vi "Lock-in_dem_mul.vi"(3 "Phase&Tc":T1(array[cluster])=[{"Phase"=-4.587448254233148, "Time constant"=0.10000000000000009, "Set TimeConstant"=FALSE, "Autophase"=FALSE, "Order"=2.0}, {"Phase"=0.0, "Time constant"=0.2, "Set TimeConstant"=FALSE, "Autophase"=FALSE, "Order"=2.0}, {"Phase"=0.0, "Time constant"=0.0, "Set TimeConstant"=FALSE, "Autophase"=FALSE, "Order"=0.0}, {"Phase"=0.0, "Time constant"=0.0, "Set TimeConstant"=FALSE, "Autophase"=FALSE, "Order"=0.0}] {"Phase" min=0.0 max=360.0 scale=0.0..360.0}, 4 "Ref in":T2(array[cluster])=[{"Ref X"=array[40000 elements], "Ref Y"=array[40000 elements], "AI Rate"=200000.0, "AI Block Size"=40000.0, "Frequency"=20.0, "Ref amp"=5.0}, {"Ref X"=array[40000 elements], "Ref Y"=array[40000 elements], "AI Rate"=200000.0, "AI Block Size"=40000.0, "Frequency"=20.0, "Ref amp"=5.0}, {"Ref X"=array[40000 elements], "Ref Y"=array[40000 elements], "AI Rate"=200000.0, "AI Block Size"=40000.0, "Frequency"=20.0, "Ref amp"=5.0}, {"Ref X"=array[40000 elements], "Ref Y"=array[40000 elements], "AI Rate"=200000.0, "AI Block Size"=40000.0, "Frequency"=20.0, "Ref amp"=5.0}] {"Ref amp" step=0.001 format="%0.4f"; "Frequency" step=0.001 format="%0.4f"; "AI Block Size" step=0.001 format="%0.4f"; "AI Rate" step=0.001 format="%0.4f"}, 5 "Signal":dbl[][](array[numeric])=array4x40000[160000 elements]) -> (1 "Demodulation":dbl[][](array[numeric])=[[0.032308985716257205, -0.0020089800684537727, 0.032371384878394444, -3.5583001590229886], [0.023385861272623584, -0.0014539178662531169, 0.02343101330770514, -3.5574201885889787], [-3.111140914765216e-05, 2.7289487058700542e-06, 3.123206852318323e-05, -5.0131650508604935], [-3.1370210865590166e-05, 3.1631661467659442e-06, 3.1532606636697875e-05, -5.751181571584788]])   [LabVIEW 2011]
uses:
  <vilib>/Analysis/3filter.llb/Filter Passband Type.ctl
  <vilib>/Analysis/NI_AALBase.lvlib
  <vilib>/ptbypt/NI_PtbyPt.lvlib
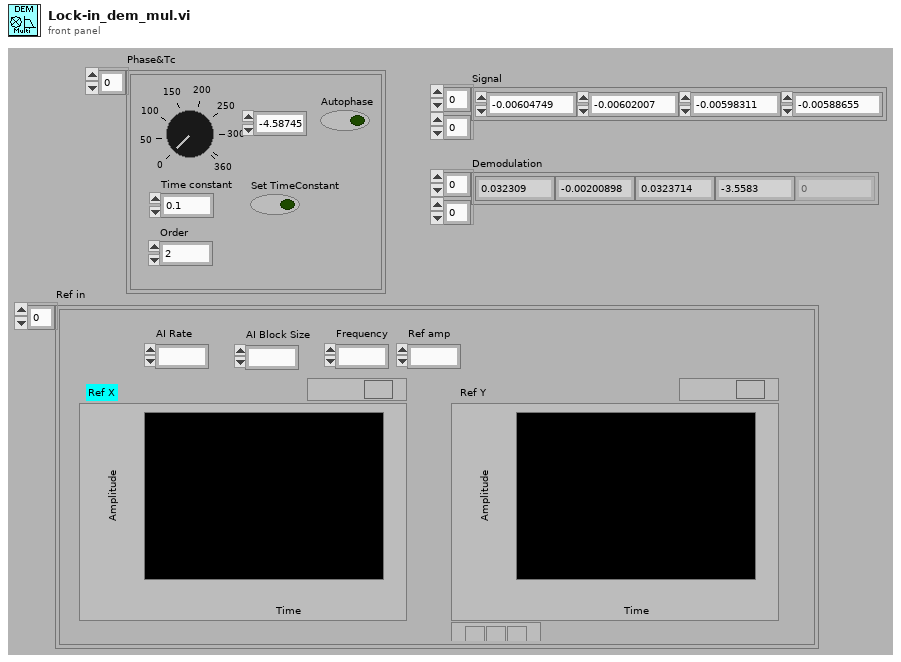
[diagram p1: front panel]
types:
  T1 = cluster{"Phase":dbl, "Time constant":dbl, "Set TimeConstant":bool, "Autophase":bool, "Order":dbl}[]
  T2 = cluster{"Ref X":dbl[], "Ref Y":dbl[], "AI Rate":dbl, "AI Block Size":dbl, "Frequency":dbl, "Ref amp":dbl}[]
  T3 = typedef "NI_AALBase.lvlib/Filter Passband Type.ctl" = enum32{"Lowpass", "Highpass", "Bandpass", "Bandstop"}
  T4 = cluster{"Ref X":dbl[], "Ref Y":dbl[], "AI Rate":dbl, "AI Block Size":dbl, "Frequency":dbl, "Ref amp":dbl}
  T5 = cluster{"Phase":dbl, "Time constant":dbl, "Set TimeConstant":bool, "Autophase":bool, "Order":dbl}
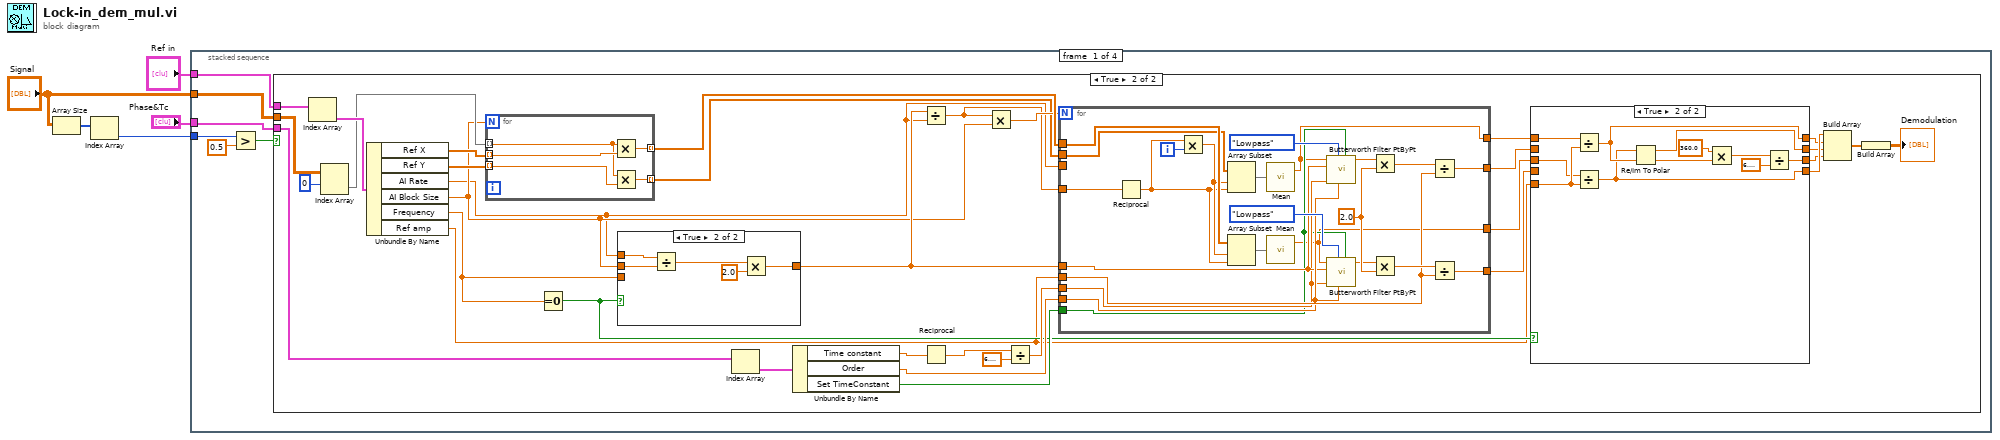
[diagram p0: block diagram]
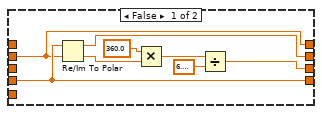
[diagram p3: hidden frame]
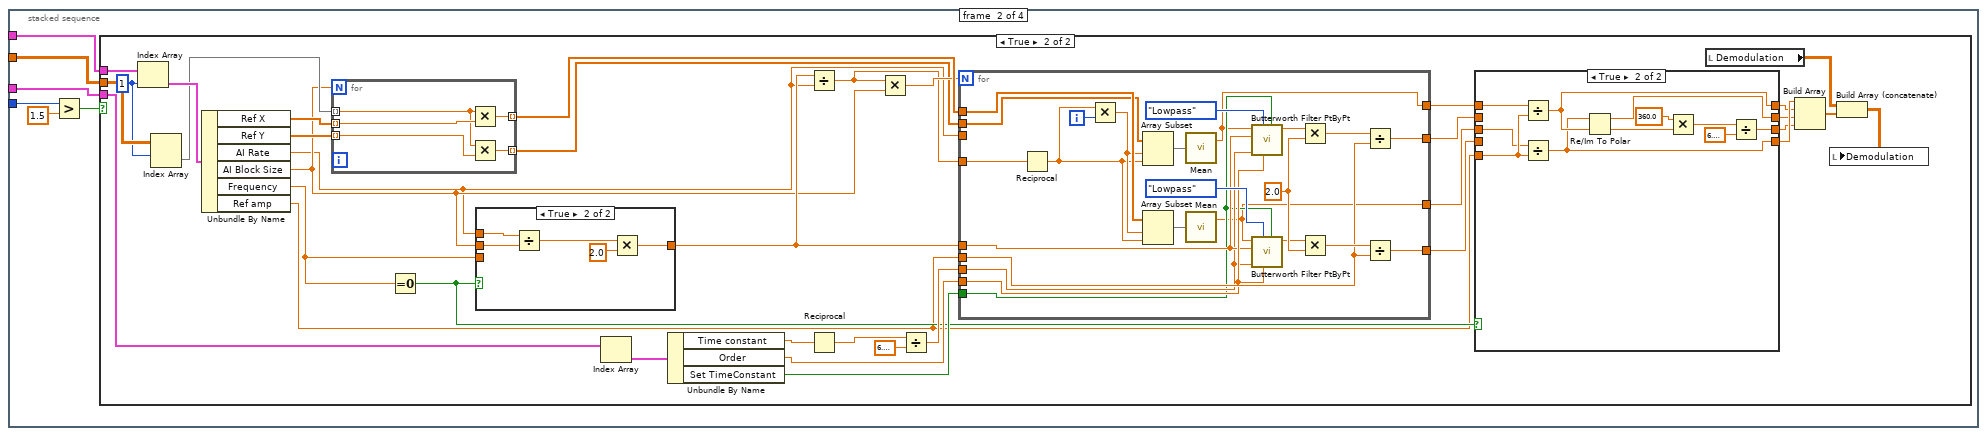
[diagram p5: hidden frame]
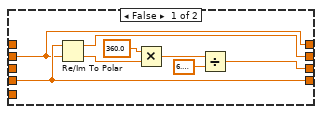
[diagram p7: hidden frame]
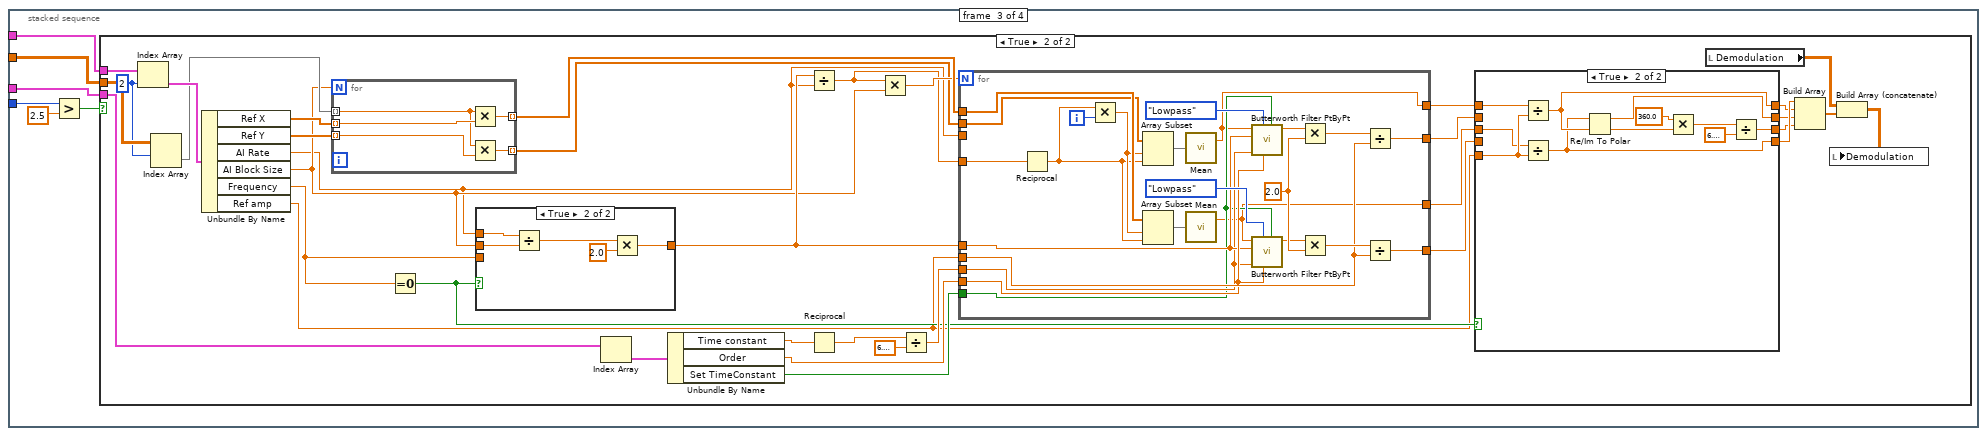
[diagram p9: hidden frame]
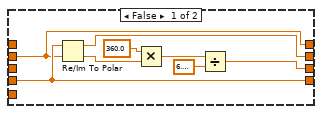
[diagram p11: hidden frame]
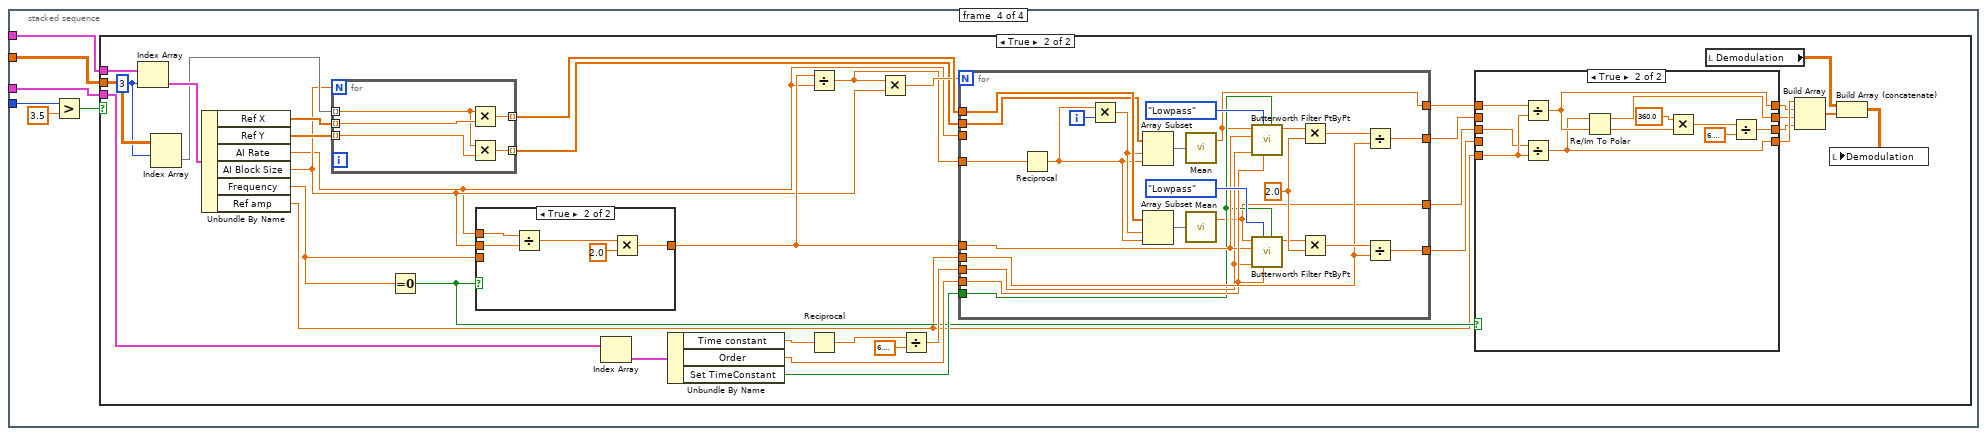
[diagram p13: hidden frame]
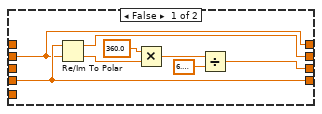
[diagram p15: hidden frame]
diagram:
  n1 = Array Size(array="Signal") -> (size(s)=w2:i32[])
  n2 = Index Array(array=w2) -> (element=w1:i32)  [unwired: 1 in]
  n3 = stacked-sequence {
    tunnel: "Signal" -> [w11 w106 w202 w298]
    tunnel: "Ref in" -> [w10 w105 w201 w297]
    tunnel: "Phase&Tc" -> [w9 w104 w200 w296]
    tunnel: w1 -> [w6 w101 w197 w293]
    frame #0 {
      n4 = Greater?(x=w6, y=0.5) -> (0:w8:bool)
      n5 = case shown="True" w8 {
        tunnel: w11 -> [_ w35]
        tunnel: w10 -> [_ w34]
        tunnel: w9 -> [_ w32]
        frame False {
        }
        frame True {
          n6 = Index Array(array=w34) -> (element=w33:T4)  [unwired: 1 in]
          n7 = Index Array(array=w35, index (row)=0) -> (element=w29:dbl[])  [unwired: 1 in]
          n8 = Unbundle By Name(w33) -> ("Ref X"=w39:dbl[], "Ref Y"=w38:dbl[], "AI Rate"=w24:dbl, "AI Block Size"=w25:dbl, "Frequency"=w27:dbl, "Ref amp"=w12:dbl)
          n9 = for {
            N: w25 -> [_]
            tunnel: w29 -> [w98] mode=indexing
            tunnel: w39 -> [w100] mode=indexing
            tunnel: [w99] -> w46 mode=indexing
            tunnel: w38 -> [w97] mode=indexing
            tunnel: [w96] -> w43 mode=indexing
            n10 = Multiply(x=w98, y=w100) -> (x*y=w99:dbl)
            n11 = Multiply(x=w98, y=w97) -> (x*y=w96:dbl)
          }
          n12 = Equal To 0?(x=w27) -> (x = 0?=w23:bool)
          n13 = case shown="True" w23 {
            tunnel: w27 -> [w66 _]
            tunnel: [w66 w67] -> w26
            tunnel: w25 -> [_ w71]
            tunnel: w24 -> [_ w70]
            frame False {
            }
            frame True {
              n14 = Divide(x=w70, y=w71) -> (x/y=w69:dbl)
              n15 = Multiply(x=w69, y=2.0) -> (x*y=w67:dbl)
            }
          }
          n16 = Index Array(array=w32) -> (element=w31:T5)  [unwired: 1 in]
          n17 = Unbundle By Name(w31) -> ("Time constant"=w37:dbl, "Order"=w36:dbl, "Set TimeConstant"=w30:bool)
          n18 = Divide(x=w26, y=w24) -> (x/y=w44:dbl)
          n19 = Reciprocal(x=w37) -> (1/x=w42:dbl)
          n20 = Multiply(x=w44, y=w25) -> (x*y=w45:dbl)
          n21 = Divide(x=w42, y=6.283185307179586) -> (x/y=w40:dbl)
          n22 = for {
            N: w45 -> [_]
            tunnel: w24 -> [_]
            tunnel: w46 -> [w95]
            tunnel: w44 -> [w88]
            tunnel: w43 -> [w93]
            tunnel: w40 -> [w78]
            tunnel: w12 -> [w81]
            tunnel: w36 -> [w80]
            tunnel: w26 -> [w79]
            tunnel: w30 -> [w77]
            tunnel: [w75] -> w22
            tunnel: [w74] -> w21
            tunnel: [w73] -> w20
            tunnel: [w72] -> w19
            i -> [w94]
            w83 = 2.0 ("y")
            n23 = Reciprocal(x=w88) -> (1/x=w91:dbl)
            n24 = Multiply(x=w91, y=w94) -> (x*y=w92:dbl)
            n25 = Array Subset(array=w93, index=w92, length=w91) -> (w89:dbl[])
            n26 = Array Subset(array=w95, index=w92, length=w91) -> (w90:dbl[])
            n27 = call <vilib>:"Mean.vi"("X"=w89) -> ("mean"=w72:dbl)  [unwired: 1 out]
            n28 = call <vilib>:"Mean.vi"("X"=w90) -> ("mean"=w73:dbl)  [unwired: 1 out]
            n29 = call <vilib>:"Butterworth Filter PtByPt.vi"("initialize"=w77, "order"=w80, "filter type"=Filter_Passband_Type."Lowpass", "low cutoff freq: fl"=w78, "sampling freq: fs"=w79, "x"=w72) -> ("Filtered x"=w84:dbl)  [unwired: 3 in, 1 out]
            n30 = call <vilib>:"Butterworth Filter PtByPt.vi"("initialize"=w77, "order"=w80, "filter type"=Filter_Passband_Type."Lowpass", "low cutoff freq: fl"=w78, "sampling freq: fs"=w79, "x"=w73) -> ("Filtered x"=w76:dbl)  [unwired: 3 in, 1 out]
            n31 = Multiply(x=w84, y=w83) -> (x*y=w82:dbl)
            n32 = Multiply(x=w76, y=w83) -> (x*y=w85:dbl)
            n33 = Divide(x=w82, y=w81) -> (x/y=w74:dbl)
            n34 = Divide(x=w85, y=w81) -> (x/y=w75:dbl)
          }
          n35 = case shown="True" w23 {
            tunnel: w22 -> [w50 _]
            tunnel: w21 -> [w49 _]
            tunnel: w20 -> [_ w58]
            tunnel: w19 -> [_ w59]
            tunnel: [w50 w56] -> w18
            tunnel: [w49 w57] -> w17
            tunnel: [w48 w62] -> w16
            tunnel: [w47 w55] -> w15
            tunnel: w12 -> [_ w60]
            frame False {
              n36 = Re/Im To Polar(2:w49, 3:w50) -> (0:w54:dbl, 1:w48:dbl)
              n37 = Multiply(x=360.0 ("y"), y=w54) -> (x*y=w51:dbl)
              n38 = Divide(x=w51, y=6.283185307179586) -> (x/y=w47:dbl)
            }
            frame True {
              n39 = Divide(x=w59, y=w60) -> (x/y=w57:dbl)
              n40 = Divide(x=w58, y=w60) -> (x/y=w56:dbl)
              n41 = Re/Im To Polar(2:w57, 3:w56) -> (0:w61:dbl, 1:w62:dbl)
              n42 = Multiply(x=360.0 ("y"), y=w61) -> (x*y=w63:dbl)
              n43 = Divide(x=w63, y=6.283185307179586) -> (x/y=w55:dbl)
            }
          }
          n44 = Build Array(w18, w17, w16, w15) -> (w14:dbl[])
          n45 = Build Array(w14) -> (→"Demodulation":dbl[][])
        }
      }
    }
    frame #1 {
      n46 = Greater?(x=w101, y=1.5) -> (0:w103:bool)
      n47 = case shown="True" w103 {
        tunnel: w106 -> [_ w131]
        tunnel: w105 -> [_ w130]
        tunnel: w104 -> [_ w128]
        frame False {
        }
        frame True {
          w109 = 1 ("index")
          n48 = Index Array(array=w130, index=w109) -> (element=w129:T4)
          n49 = Index Array(array=w131, index (row)=w109) -> (element=w125:dbl[])  [unwired: 1 in]
          n50 = Unbundle By Name(w129) -> ("Ref X"=w135:dbl[], "Ref Y"=w134:dbl[], "AI Rate"=w121:dbl, "AI Block Size"=w122:dbl, "Frequency"=w124:dbl, "Ref amp"=w110:dbl)
          n51 = for {
            N: w122 -> [_]
            tunnel: w125 -> [w194] mode=indexing
            tunnel: w135 -> [w196] mode=indexing
            tunnel: [w195] -> w142 mode=indexing
            tunnel: w134 -> [w193] mode=indexing
            tunnel: [w192] -> w139 mode=indexing
            n52 = Multiply(x=w194, y=w196) -> (x*y=w195:dbl)
            n53 = Multiply(x=w194, y=w193) -> (x*y=w192:dbl)
          }
          n54 = Equal To 0?(x=w124) -> (x = 0?=w120:bool)
          n55 = case shown="True" w120 {
            tunnel: w124 -> [w162 _]
            tunnel: [w162 w163] -> w123
            tunnel: w122 -> [_ w167]
            tunnel: w121 -> [_ w166]
            frame False {
            }
            frame True {
              n56 = Divide(x=w166, y=w167) -> (x/y=w165:dbl)
              n57 = Multiply(x=w165, y=2.0) -> (x*y=w163:dbl)
            }
          }
          n58 = Index Array(array=w128) -> (element=w127:T5)  [unwired: 1 in]
          n59 = Unbundle By Name(w127) -> ("Time constant"=w133:dbl, "Order"=w132:dbl, "Set TimeConstant"=w126:bool)
          n60 = Divide(x=w123, y=w121) -> (x/y=w140:dbl)
          n61 = Reciprocal(x=w133) -> (1/x=w138:dbl)
          n62 = Multiply(x=w140, y=w122) -> (x*y=w141:dbl)
          n63 = Divide(x=w138, y=6.283185307179586) -> (x/y=w136:dbl)
          n64 = for {
            N: w141 -> [_]
            tunnel: w121 -> [_]
            tunnel: w142 -> [w191]
            tunnel: w140 -> [w184]
            tunnel: w139 -> [w189]
            tunnel: w136 -> [w174]
            tunnel: w110 -> [w177]
            tunnel: w132 -> [w176]
            tunnel: w123 -> [w175]
            tunnel: w126 -> [w173]
            tunnel: [w171] -> w119
            tunnel: [w170] -> w118
            tunnel: [w169] -> w117
            tunnel: [w168] -> w116
            i -> [w190]
            w179 = 2.0 ("y")
            n65 = Reciprocal(x=w184) -> (1/x=w187:dbl)
            n66 = Multiply(x=w187, y=w190) -> (x*y=w188:dbl)
            n67 = Array Subset(array=w189, index=w188, length=w187) -> (w185:dbl[])
            n68 = Array Subset(array=w191, index=w188, length=w187) -> (w186:dbl[])
            n69 = call <vilib>:"Mean.vi"("X"=w185) -> ("mean"=w168:dbl)  [unwired: 1 out]
            n70 = call <vilib>:"Mean.vi"("X"=w186) -> ("mean"=w169:dbl)  [unwired: 1 out]
            n71 = call <vilib>:"Butterworth Filter PtByPt.vi"("initialize"=w173, "order"=w176, "filter type"=Filter_Passband_Type."Lowpass", "low cutoff freq: fl"=w174, "sampling freq: fs"=w175, "x"=w168) -> ("Filtered x"=w180:dbl)  [unwired: 3 in, 1 out]
            n72 = call <vilib>:"Butterworth Filter PtByPt.vi"("initialize"=w173, "order"=w176, "filter type"=Filter_Passband_Type."Lowpass", "low cutoff freq: fl"=w174, "sampling freq: fs"=w175, "x"=w169) -> ("Filtered x"=w172:dbl)  [unwired: 3 in, 1 out]
            n73 = Multiply(x=w180, y=w179) -> (x*y=w178:dbl)
            n74 = Multiply(x=w172, y=w179) -> (x*y=w181:dbl)
            n75 = Divide(x=w178, y=w177) -> (x/y=w170:dbl)
            n76 = Divide(x=w181, y=w177) -> (x/y=w171:dbl)
          }
          n77 = case shown="True" w120 {
            tunnel: w119 -> [w146 _]
            tunnel: w118 -> [w145 _]
            tunnel: w117 -> [_ w154]
            tunnel: w116 -> [_ w155]
            tunnel: [w146 w152] -> w115
            tunnel: [w145 w153] -> w114
            tunnel: [w144 w158] -> w113
            tunnel: [w143 w151] -> w112
            tunnel: w110 -> [_ w156]
            frame False {
              n78 = Re/Im To Polar(2:w145, 3:w146) -> (0:w150:dbl, 1:w144:dbl)
              n79 = Multiply(x=360.0 ("y"), y=w150) -> (x*y=w147:dbl)
              n80 = Divide(x=w147, y=6.283185307179586) -> (x/y=w143:dbl)
            }
            frame True {
              n81 = Divide(x=w155, y=w156) -> (x/y=w153:dbl)
              n82 = Divide(x=w154, y=w156) -> (x/y=w152:dbl)
              n83 = Re/Im To Polar(2:w153, 3:w152) -> (0:w157:dbl, 1:w158:dbl)
              n84 = Multiply(x=360.0 ("y"), y=w157) -> (x*y=w159:dbl)
              n85 = Divide(x=w159, y=6.283185307179586) -> (x/y=w151:dbl)
            }
          }
          n86 = local read "Demodulation"() -> (w108:dbl[][])
          n87 = Build Array(w115, w114, w113, w112) -> (w111:dbl[])
          n88 = Build Array (concatenate)(w108, w111) -> (w107:dbl[][])
          n89 = local write "Demodulation"(w107) -> ()
        }
      }
    }
    frame #2 {
      n90 = Greater?(x=w197, y=2.5) -> (0:w199:bool)
      n91 = case shown="True" w199 {
        tunnel: w202 -> [_ w227]
        tunnel: w201 -> [_ w226]
        tunnel: w200 -> [_ w224]
        frame False {
        }
        frame True {
          w205 = 2 ("index")
          n92 = Index Array(array=w226, index=w205) -> (element=w225:T4)
          n93 = Index Array(array=w227, index (row)=w205) -> (element=w221:dbl[])  [unwired: 1 in]
          n94 = Unbundle By Name(w225) -> ("Ref X"=w231:dbl[], "Ref Y"=w230:dbl[], "AI Rate"=w217:dbl, "AI Block Size"=w218:dbl, "Frequency"=w220:dbl, "Ref amp"=w206:dbl)
          n95 = for {
            N: w218 -> [_]
            tunnel: w221 -> [w290] mode=indexing
            tunnel: w231 -> [w292] mode=indexing
            tunnel: [w291] -> w238 mode=indexing
            tunnel: w230 -> [w289] mode=indexing
            tunnel: [w288] -> w235 mode=indexing
            n96 = Multiply(x=w290, y=w292) -> (x*y=w291:dbl)
            n97 = Multiply(x=w290, y=w289) -> (x*y=w288:dbl)
          }
          n98 = Equal To 0?(x=w220) -> (x = 0?=w216:bool)
          n99 = case shown="True" w216 {
            tunnel: w220 -> [w258 _]
            tunnel: [w258 w259] -> w219
            tunnel: w218 -> [_ w263]
            tunnel: w217 -> [_ w262]
            frame False {
            }
            frame True {
              n100 = Divide(x=w262, y=w263) -> (x/y=w261:dbl)
              n101 = Multiply(x=w261, y=2.0) -> (x*y=w259:dbl)
            }
          }
          n102 = Index Array(array=w224) -> (element=w223:T5)  [unwired: 1 in]
          n103 = Unbundle By Name(w223) -> ("Time constant"=w229:dbl, "Order"=w228:dbl, "Set TimeConstant"=w222:bool)
          n104 = Divide(x=w219, y=w217) -> (x/y=w236:dbl)
          n105 = Reciprocal(x=w229) -> (1/x=w234:dbl)
          n106 = Multiply(x=w236, y=w218) -> (x*y=w237:dbl)
          n107 = Divide(x=w234, y=6.283185307179586) -> (x/y=w232:dbl)
          n108 = for {
            N: w237 -> [_]
            tunnel: w217 -> [_]
            tunnel: w238 -> [w287]
            tunnel: w236 -> [w280]
            tunnel: w235 -> [w285]
            tunnel: w232 -> [w270]
            tunnel: w206 -> [w273]
            tunnel: w228 -> [w272]
            tunnel: w219 -> [w271]
            tunnel: w222 -> [w269]
            tunnel: [w267] -> w215
            tunnel: [w266] -> w214
            tunnel: [w265] -> w213
            tunnel: [w264] -> w212
            i -> [w286]
            w275 = 2.0 ("y")
            n109 = Reciprocal(x=w280) -> (1/x=w283:dbl)
            n110 = Multiply(x=w283, y=w286) -> (x*y=w284:dbl)
            n111 = Array Subset(array=w285, index=w284, length=w283) -> (w281:dbl[])
            n112 = Array Subset(array=w287, index=w284, length=w283) -> (w282:dbl[])
            n113 = call <vilib>:"Mean.vi"("X"=w281) -> ("mean"=w264:dbl)  [unwired: 1 out]
            n114 = call <vilib>:"Mean.vi"("X"=w282) -> ("mean"=w265:dbl)  [unwired: 1 out]
            n115 = call <vilib>:"Butterworth Filter PtByPt.vi"("initialize"=w269, "order"=w272, "filter type"=Filter_Passband_Type."Lowpass", "low cutoff freq: fl"=w270, "sampling freq: fs"=w271, "x"=w264) -> ("Filtered x"=w276:dbl)  [unwired: 3 in, 1 out]
            n116 = call <vilib>:"Butterworth Filter PtByPt.vi"("initialize"=w269, "order"=w272, "filter type"=Filter_Passband_Type."Lowpass", "low cutoff freq: fl"=w270, "sampling freq: fs"=w271, "x"=w265) -> ("Filtered x"=w268:dbl)  [unwired: 3 in, 1 out]
            n117 = Multiply(x=w276, y=w275) -> (x*y=w274:dbl)
            n118 = Multiply(x=w268, y=w275) -> (x*y=w277:dbl)
            n119 = Divide(x=w274, y=w273) -> (x/y=w266:dbl)
            n120 = Divide(x=w277, y=w273) -> (x/y=w267:dbl)
          }
          n121 = case shown="True" w216 {
            tunnel: w215 -> [w242 _]
            tunnel: w214 -> [w241 _]
            tunnel: w213 -> [_ w250]
            tunnel: w212 -> [_ w251]
            tunnel: [w242 w248] -> w211
            tunnel: [w241 w249] -> w210
            tunnel: [w240 w254] -> w209
            tunnel: [w239 w247] -> w208
            tunnel: w206 -> [_ w252]
            frame False {
              n122 = Re/Im To Polar(2:w241, 3:w242) -> (0:w246:dbl, 1:w240:dbl)
              n123 = Multiply(x=360.0 ("y"), y=w246) -> (x*y=w243:dbl)
              n124 = Divide(x=w243, y=6.283185307179586) -> (x/y=w239:dbl)
            }
            frame True {
              n125 = Divide(x=w251, y=w252) -> (x/y=w249:dbl)
              n126 = Divide(x=w250, y=w252) -> (x/y=w248:dbl)
              n127 = Re/Im To Polar(2:w249, 3:w248) -> (0:w253:dbl, 1:w254:dbl)
              n128 = Multiply(x=360.0 ("y"), y=w253) -> (x*y=w255:dbl)
              n129 = Divide(x=w255, y=6.283185307179586) -> (x/y=w247:dbl)
            }
          }
          n130 = local read "Demodulation"() -> (w204:dbl[][])
          n131 = Build Array(w211, w210, w209, w208) -> (w207:dbl[])
          n132 = Build Array (concatenate)(w204, w207) -> (w203:dbl[][])
          n133 = local write "Demodulation"(w203) -> ()
        }
      }
    }
    frame #3 {
      n134 = Greater?(x=w293, y=3.5) -> (0:w295:bool)
      n135 = case shown="True" w295 {
        tunnel: w298 -> [_ w323]
        tunnel: w297 -> [_ w322]
        tunnel: w296 -> [_ w320]
        frame False {
        }
        frame True {
          w301 = 3 ("index")
          n136 = Index Array(array=w322, index=w301) -> (element=w321:T4)
          n137 = Index Array(array=w323, index (row)=w301) -> (element=w317:dbl[])  [unwired: 1 in]
          n138 = Unbundle By Name(w321) -> ("Ref X"=w327:dbl[], "Ref Y"=w326:dbl[], "AI Rate"=w313:dbl, "AI Block Size"=w314:dbl, "Frequency"=w316:dbl, "Ref amp"=w302:dbl)
          n139 = for {
            N: w314 -> [_]
            tunnel: w317 -> [w386] mode=indexing
            tunnel: w327 -> [w388] mode=indexing
            tunnel: [w387] -> w334 mode=indexing
            tunnel: w326 -> [w385] mode=indexing
            tunnel: [w384] -> w331 mode=indexing
            n140 = Multiply(x=w386, y=w388) -> (x*y=w387:dbl)
            n141 = Multiply(x=w386, y=w385) -> (x*y=w384:dbl)
          }
          n142 = Equal To 0?(x=w316) -> (x = 0?=w312:bool)
          n143 = case shown="True" w312 {
            tunnel: w316 -> [w354 _]
            tunnel: [w354 w355] -> w315
            tunnel: w314 -> [_ w359]
            tunnel: w313 -> [_ w358]
            frame False {
            }
            frame True {
              n144 = Divide(x=w358, y=w359) -> (x/y=w357:dbl)
              n145 = Multiply(x=w357, y=2.0) -> (x*y=w355:dbl)
            }
          }
          n146 = Index Array(array=w320) -> (element=w319:T5)  [unwired: 1 in]
          n147 = Unbundle By Name(w319) -> ("Time constant"=w325:dbl, "Order"=w324:dbl, "Set TimeConstant"=w318:bool)
          n148 = Divide(x=w315, y=w313) -> (x/y=w332:dbl)
          n149 = Reciprocal(x=w325) -> (1/x=w330:dbl)
          n150 = Multiply(x=w332, y=w314) -> (x*y=w333:dbl)
          n151 = Divide(x=w330, y=6.283185307179586) -> (x/y=w328:dbl)
          n152 = for {
            N: w333 -> [_]
            tunnel: w313 -> [_]
            tunnel: w334 -> [w383]
            tunnel: w332 -> [w376]
            tunnel: w331 -> [w381]
            tunnel: w328 -> [w366]
            tunnel: w302 -> [w369]
            tunnel: w324 -> [w368]
            tunnel: w315 -> [w367]
            tunnel: w318 -> [w365]
            tunnel: [w363] -> w311
            tunnel: [w362] -> w310
            tunnel: [w361] -> w309
            tunnel: [w360] -> w308
            i -> [w382]
            w371 = 2.0 ("y")
            n153 = Reciprocal(x=w376) -> (1/x=w379:dbl)
            n154 = Multiply(x=w379, y=w382) -> (x*y=w380:dbl)
            n155 = Array Subset(array=w381, index=w380, length=w379) -> (w377:dbl[])
            n156 = Array Subset(array=w383, index=w380, length=w379) -> (w378:dbl[])
            n157 = call <vilib>:"Mean.vi"("X"=w377) -> ("mean"=w360:dbl)  [unwired: 1 out]
            n158 = call <vilib>:"Mean.vi"("X"=w378) -> ("mean"=w361:dbl)  [unwired: 1 out]
            n159 = call <vilib>:"Butterworth Filter PtByPt.vi"("initialize"=w365, "order"=w368, "filter type"=Filter_Passband_Type."Lowpass", "low cutoff freq: fl"=w366, "sampling freq: fs"=w367, "x"=w360) -> ("Filtered x"=w372:dbl)  [unwired: 3 in, 1 out]
            n160 = call <vilib>:"Butterworth Filter PtByPt.vi"("initialize"=w365, "order"=w368, "filter type"=Filter_Passband_Type."Lowpass", "low cutoff freq: fl"=w366, "sampling freq: fs"=w367, "x"=w361) -> ("Filtered x"=w364:dbl)  [unwired: 3 in, 1 out]
            n161 = Multiply(x=w372, y=w371) -> (x*y=w370:dbl)
            n162 = Multiply(x=w364, y=w371) -> (x*y=w373:dbl)
            n163 = Divide(x=w370, y=w369) -> (x/y=w362:dbl)
            n164 = Divide(x=w373, y=w369) -> (x/y=w363:dbl)
          }
          n165 = case shown="True" w312 {
            tunnel: w311 -> [w338 _]
            tunnel: w310 -> [w337 _]
            tunnel: w309 -> [_ w346]
            tunnel: w308 -> [_ w347]
            tunnel: [w338 w344] -> w307
            tunnel: [w337 w345] -> w306
            tunnel: [w336 w350] -> w305
            tunnel: [w335 w343] -> w304
            tunnel: w302 -> [_ w348]
            frame False {
              n166 = Re/Im To Polar(2:w337, 3:w338) -> (0:w342:dbl, 1:w336:dbl)
              n167 = Multiply(x=360.0 ("y"), y=w342) -> (x*y=w339:dbl)
              n168 = Divide(x=w339, y=6.283185307179586) -> (x/y=w335:dbl)
            }
            frame True {
              n169 = Divide(x=w347, y=w348) -> (x/y=w345:dbl)
              n170 = Divide(x=w346, y=w348) -> (x/y=w344:dbl)
              n171 = Re/Im To Polar(2:w345, 3:w344) -> (0:w349:dbl, 1:w350:dbl)
              n172 = Multiply(x=360.0 ("y"), y=w349) -> (x*y=w351:dbl)
              n173 = Divide(x=w351, y=6.283185307179586) -> (x/y=w343:dbl)
            }
          }
          n174 = local read "Demodulation"() -> (w300:dbl[][])
          n175 = Build Array(w307, w306, w305, w304) -> (w303:dbl[])
          n176 = Build Array (concatenate)(w300, w303) -> (w299:dbl[][])
          n177 = local write "Demodulation"(w299) -> ()
        }
      }
    }
  }
